vi "Set VI Help from Help Info File (Simple).vi"(6 "Link to HTML (F)":bool, 8 "error in":errorcluster, 9 "Save Params":T2, 10 "Build Params":T3={"Help Targeting"=enum."relative", "Subfolder"="", "CHM Tag mode"=enum."HTML Filename"}, 11 "Help Info File":path) -> (0 "error out":errorcluster, 1 "Source Files Help Info":T1(array[cluster]), 2 "Source File Paths":path[](array[path]), 3 "dup Help Info File":path)   [LabVIEW 2014, in "VIHelpeksAPI.lvlib"]
doc: "The VI reads the <b>Help Info File</b> generated by VI Helpeks during help generation and returns information on the source files and details on their help links according to the input parameters. In addition, if enabled, the VI applies the help information to the source VIs and palettes (.mnu files).\n\nThe <b>Example VI</b> demonstrating the use of VIHelpeks API can be opened using the \"Tools >> VI Helpeks >> Help and Support\" menu. Alternatively, you can launch the <b>NI Example Finder</b> and search for \"VI Helpeks\", or find it within the <b><labview>\\Examples\\VI Helpeks</b> folder.\n\n::: VI Helpeks :::\nCopyright (c) 2000-2026 Konstantin Shifershteyn. All rights reserved."
uses:
  VIHelpeksAPI.lvlib
panel:
  # "VI Helpeks\nCopyright (c) 2012-2026 Konstantin Shifershteyn"
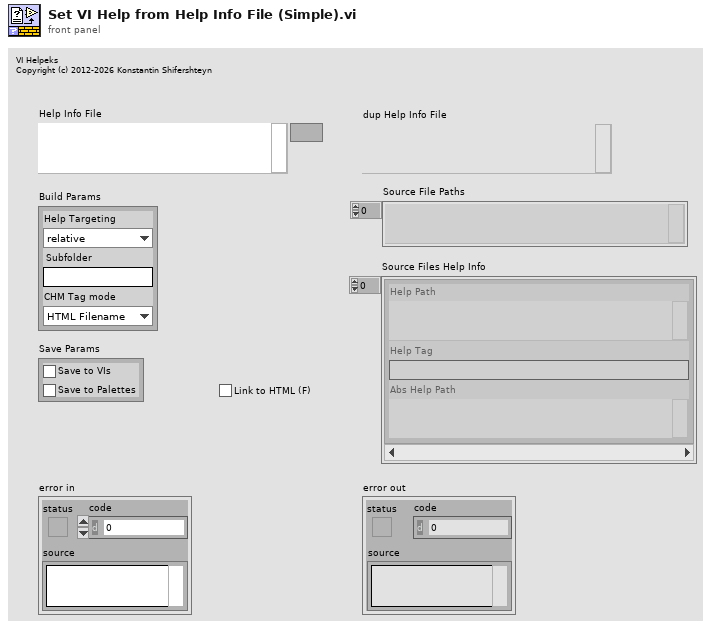
[diagram p1: front panel]
types:
  T1 = cluster{"Help Path":path, "Help Tag":string, "Abs Help Path":path}[]
  T2 = cluster{"Save to VIs":bool, "Save to Palettes":bool}
  T3 = cluster{"Help Targeting":enum16{"absolute", "relative", "<helpdir>", "<userlib>", "<vilib>", "<instrlib>"}, "Subfolder":string, "CHM Tag mode":enum16{"HTML Filename", "Index Keyword"}}
  T4 = cluster{"Source File Name":string, "Source File Path":path, "HTML File Path":path, "CHM Local Path":string, "CHM Keyword":string}[]
  T5 = cluster{"HHP File":path, "TOC File":path, "IDX File":path, "CHM File":path}
  T6 = enum16{"absolute", "relative", "<helpdir>", "<userlib>", "<vilib>", "<instrlib>"}
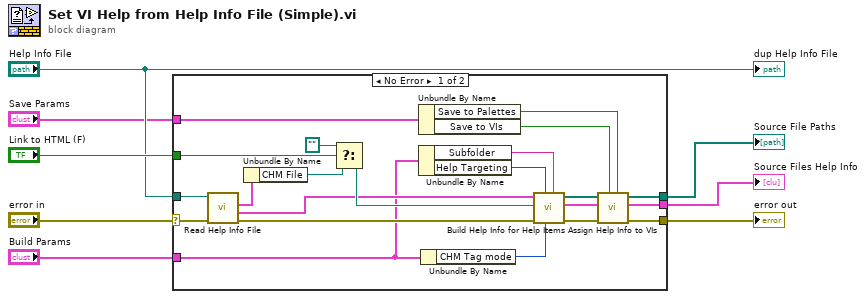
[diagram p0: block diagram]
diagram:
  n1 = case shown="No Error" "error in" {
    selector: "error in" -> [w9 w31]
    tunnel: "Link to HTML (F)" -> [w29 _]
    tunnel: [w20 w31] -> w7
    tunnel: "Help Info File" -> [w19 _]
    tunnel: "Save Params" -> [w18 _]
    tunnel: "Build Params" -> [w14 _]
    tunnel: [w11 _] -> w3
    tunnel: [w10 _] -> w2
    frame No Error {
      n2 = call "Read Help Info File.vi"("error in"=w9, "Help Info File"=w19) -> ("error out"=w30:errorcluster, "Help Items"=w24:T4, "Help Paths"=w28:T5)  [unwired: 6 in, 1 out]
      n3 = Unbundle By Name(w28) -> ("CHM File"=w27:path)
      n4 = Select(t=path "", s=w29, f=w27) -> (s? t:f=w25:path)
      n5 = Unbundle By Name(w18) -> ("Save to Palettes"=w16:bool, "Save to VIs"=w17:bool)
      n6 = Unbundle By Name(w14) -> ("Subfolder"=w12:string, "Help Targeting"=w13:T6)
      n7 = Unbundle By Name(w14) -> ("CHM Tag mode"=w15:enum16{"HTML Filename", "Index Keyword"})
      n8 = call "Build Help Info for Help Items.vi"("Subfolder"=w12, "CHM Tag mode"=w15, "Help Targeting"=w13, "error in"=w30, "CHM File (empty)"=w25, "Help Items"=w24) -> ("error out"=w23:errorcluster, "Source Files Help Info"=w21:T1, "Source File Paths"=w22:path[])  [unwired: 3 in]
      n9 = call "Assign Help Info to VIs.vi"("Save to Palettes (T)"=w16, "Save to VIs (T)"=w17, "error in"=w23, "Source Files Help Info"=w21, "Source File Paths"=w22) -> ("error out"=w20:errorcluster, "dup Source Files Help Info"=w11:T1, "dup Source File Paths"=w10:path[])  [unwired: 4 in]
    }
    frame Error {
    }
  }
  "error out" <- w7
  "Source Files Help Info" <- w3
  "Source File Paths" <- w2
  "dup Help Info File" <- "Help Info File"
